vi "Get NamedBundler Input.vi"(8 "error in (no error)":errorcluster, 10 "Input name":string, 11 "NamedBundler ref in":refnum<vi>) -> (0 "error out":errorcluster, 1 "Found?":bool, 2 "Input Term ref":refnum<vi>, 3 "NamedBundler ref out":refnum<vi>)   [LabVIEW 2019, in "gRPC Template Creation Utility.lvlib"]
uses:
  gRPC Template Creation Utility.lvlib
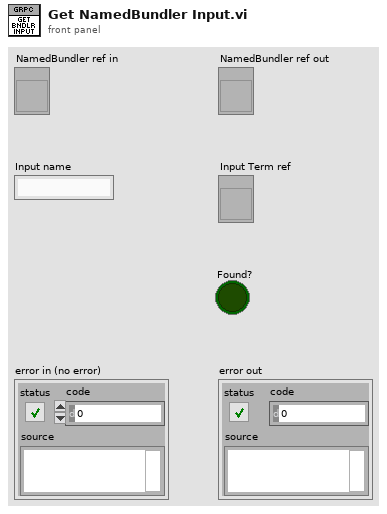
[diagram p1: front panel]
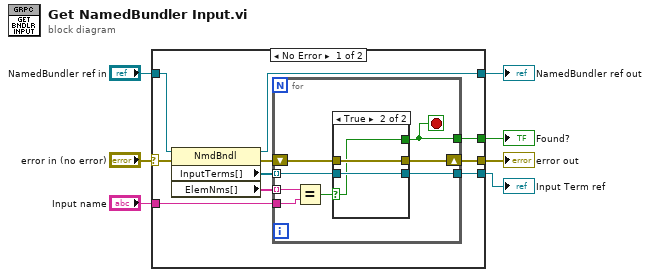
[diagram p0: block diagram]
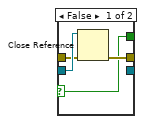
[diagram p2: hidden frame]
diagram:
  n1 = case shown="No Error" "error in (no error)" {
    selector: "error in (no error)" -> [w10 w34]
    tunnel: "Input name" -> [w17 _]
    tunnel: [w8 w34] -> w6
    tunnel: "NamedBundler ref in" -> [w13 w33]
    tunnel: [w14 _] -> w3
    tunnel: [w11 w33] -> w2
    tunnel: [w12 _] -> w1
    frame No Error {
      n2 = property class="NmdBndl"(reference=w13, error in=w10) -> (reference out=w11:refnum<vi>, error out=w9:errorcluster, "InputTerms[]"=w15:refnum<vi>[], "ElemNms[]"=w16:string[])
      n3 = for {
        tunnel: w17 -> [w25]
        tunnel: [w20] -> w12
        tunnel: w16 -> [w23] mode=indexing
        tunnel: w15 -> [w22] mode=indexing
        tunnel: [w21] -> w14
        shift-right: [w18] -> w8
        shift-left: w9 -> [w19]
        stop <- w20 stop-if-true
        n4 = Equal?(x=w23, y=w25) -> (x = y?=w24:bool)
        n5 = case shown="True" w24 {
          selector: w24 -> [w26 w30]
          tunnel: [w26 w30] -> w20
          tunnel: w22 -> [w29 w32]
          tunnel: [_ w32] -> w21
          tunnel: w19 -> [w28 w31]
          tunnel: [w27 w31] -> w18
          frame False {
            n6 = Close Reference(reference=w29, error in (no error)=w28) -> (error out=w27:errorcluster)
          }
          frame True {
          }
        }
      }
    }
    frame Error {
    }
  }
  "error out" <- w6
  "NamedBundler ref out" <- w2
  "Input Term ref" <- w3
  "Found?" <- w1
